vi "Offset Measurement Accumulate.vi"(8 "error in (no error)":errorcluster, 9 "DC":dbl[](array[numeric]), 10 "Offset Measurement":T1={"phase"=enum."idle", "measureInputOffset"={"buffers"=0, "settle"=2, "timeout"=5.0, "channels"=[], "zero"=enum."both"}, "settle remaining"=0, "buffers remaining"=0, "deadline"=0, "sum"=[], "count"=0, "saved amplitudes"=[], "saved offsets"=[], "previous status"=enum."created"}, 11 "Instrument.DAQ in":refnum<class "Instrument.DAQ.lvclass">) -> (0 "error out":errorcluster, 2 "Offset Measurement":T1={"phase"=enum."idle", "measureInputOffset"={"buffers"=0, "settle"=2, "timeout"=5.0, "channels"=[], "zero"=enum."both"}, "settle remaining"=0, "buffers remaining"=0, "deadline"=0, "sum"=[], "count"=0, "saved amplitudes"=[], "saved offsets"=[], "previous status"=enum."created"}, 3 "Instrument.DAQ out":refnum<class "Instrument.DAQ.lvclass">)   [LabVIEW 2019, in "Instrument.Lockin.lvlib" / "Instrument.DAQ.lvclass"]
uses:
  Instrument.DAQ.lvclass
  Typedefs/Offset Measurement--Cluster.ctl
  Lockin.Typedefs/API/Lockin.measureInputOffset Config--Cluster.ctl
  Lockin.Typedefs/API/Lockin.measureInputOffset.zero--enum.ctl
  Lockin.Typedefs/other/Status--enum.ctl
  Lockin.Typedefs/Lockin.Typedefs.lvlib
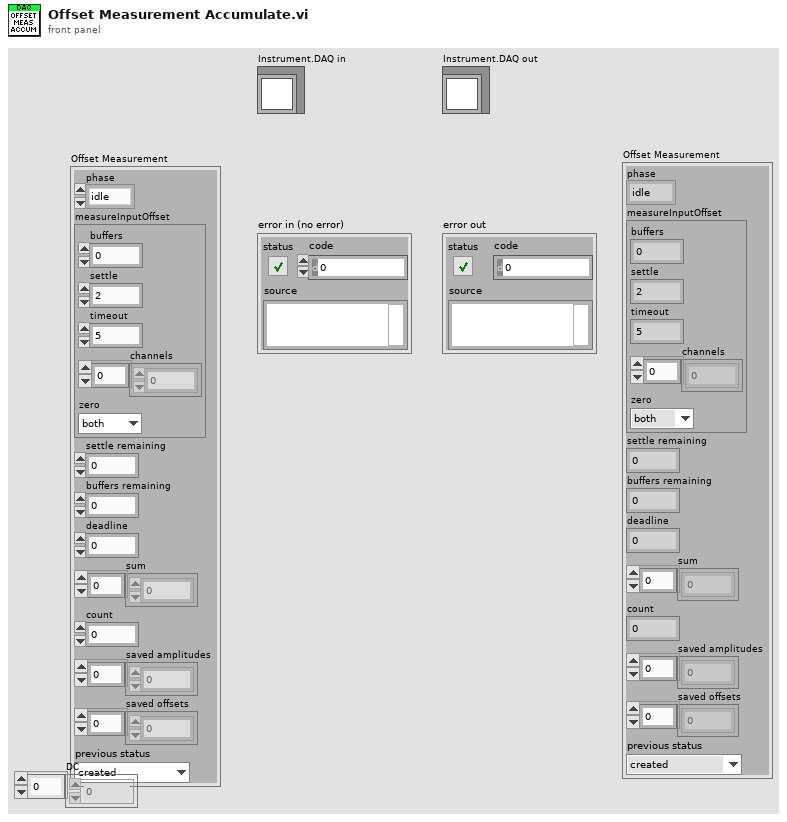
[diagram p1: front panel]
types:
  T1 = typedef "Instrument.Lockin.lvlib/Instrument.DAQ.lvclass/Offset Measurement--Cluster.ctl" = cluster{"phase":enum16{"idle", "zeroing", "settling", "averaging", "done", "aborted", "cancelled", "timed out"}, "measureInputOffset":T2, "settle remaining":i32, "buffers remaining":i32, "deadline":u32, "sum":dbl[], "count":i32, "saved amplitudes":dbl[], "saved offsets":dbl[], "previous status":T4}
  T2 = typedef "Lockin.Typedefs.lvlib/Lockin.measureInputOffset Config--Cluster.ctl" = cluster{"buffers":i32, "settle":i32, "timeout":dbl, "channels":i32[], "zero":T3}
  T3 = typedef "Lockin.Typedefs.lvlib/Lockin.measureInputOffset.zero--enum.ctl" = enum16{"both", "ac", "dc", "none"}
  T4 = typedef "Lockin.Typedefs.lvlib/Status--enum.ctl" = enum16{"idle", "created", "started", "stopped", "sweeping", "measuring offset"}
  T5 = enum16{"idle", "zeroing", "settling", "averaging", "done", "aborted", "cancelled", "timed out"}
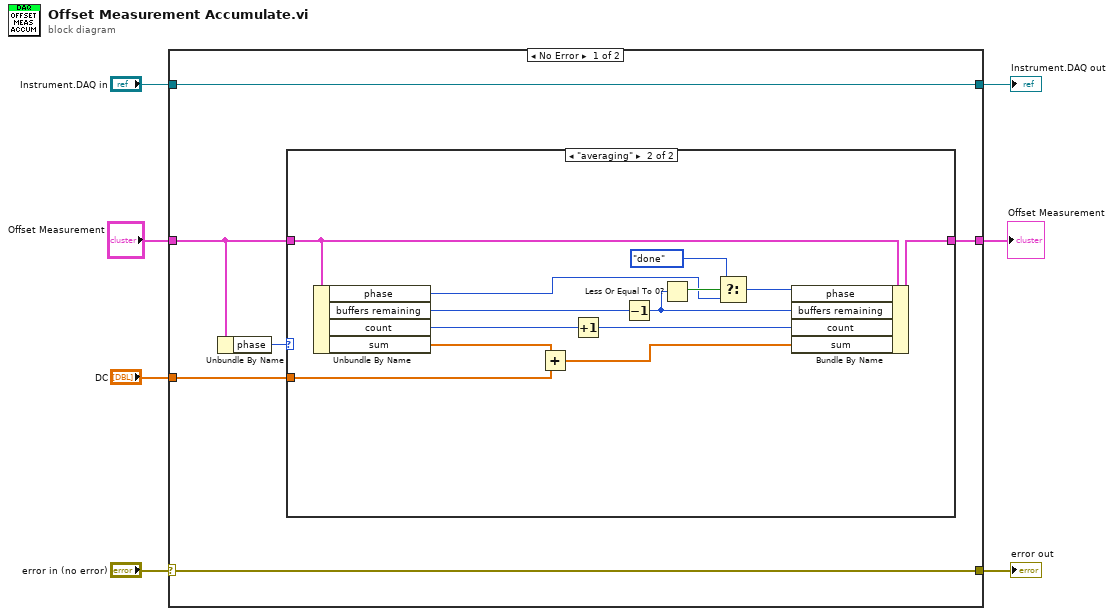
[diagram p0: block diagram]
diagram:
  n1 = case shown="No Error" "error in (no error)" {
    selector: "error in (no error)" -> [w9 w30]
    tunnel: "Offset Measurement" -> [w13 w28]
    tunnel: [w12 w28] -> w6
    tunnel: "DC" -> [w10 _]
    tunnel: [w9 w30] -> w3
    tunnel: [w8 w29] -> w2
    tunnel: "Instrument.DAQ in" -> [w8 w29]
    frame No Error {
      n2 = Unbundle By Name(w13) -> ("phase"=w11:T5)
      n3 = case shown="\"averaging\"" w11 {
        tunnel: w13 -> [w14 w23]
        tunnel: [w14 w24] -> w12
        tunnel: w10 -> [_ w26]
        frame Default {
        }
        frame "averaging" {
          n4 = Unbundle By Name(w23) -> ("phase"=w16:T5, "buffers remaining"=w20:i32, "count"=w22:i32, "sum"=w27:dbl[])
          n5 = Add(x=w27, y=w26) -> (x+y=w25:dbl[])
          n6 = Increment(x=w22) -> (x+1=w21:i32)
          n7 = Decrement(x=w20) -> (x-1=w19:i32)
          n8 = Less Or Equal To 0?(x=w19) -> (x <= 0?=w18:bool)
          n9 = Select(t=T5."done", s=w18, f=w16) -> (s? t:f=w17:T5)
          n10 = Bundle By Name(cluster=w23, "phase"=w17, "buffers remaining"=w19, "count"=w21, "sum"=w25) -> (w24:T1)
        }
      }
    }
    frame Error {
    }
  }
  "error out" <- w3
  "Instrument.DAQ out" <- w2
  "Offset Measurement" <- w6
